vi "Main - Auto Detect Modules.vi"(8 "error in (no error)":errorcluster, 11 "Node Ptr":u64 format="%.0x") -> (0 "error out":errorcluster)   [LabVIEW 2020, in "SEECD System Explorer.lvlib"]
uses:
  SEECD System Explorer.lvlib
  Shared/Globals/String Constants.vi
  Shared/Globals/Scan Engine GUIDs.vi
  Shared/Globals/Property Strings.vi
  <vilib>/NI VeriStand/Custom Device API/Custom Device API.lvlib
  Shared/SEECD Shared.lvlib
  Scripting/Scan Engine Scripting.lvlib
panel:
  in  "Tag":string
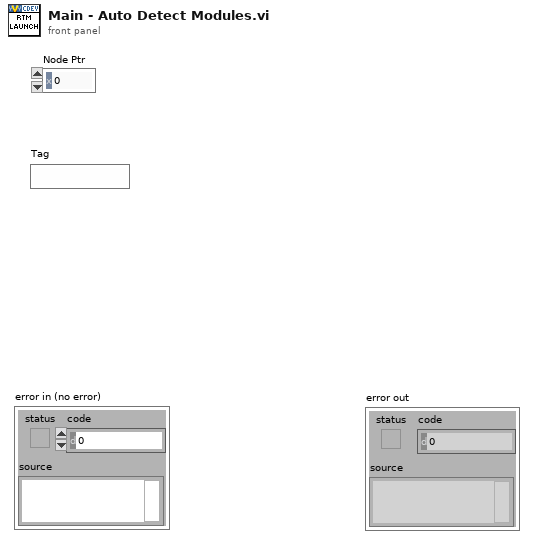
[diagram p1: front panel]
types:
  T1 = typedef "Custom Device API.lvlib/Custom Device Item Ref.ctl" = u64
  T2 = typedef "SEECD System Explorer.lvlib/Slot Programming Mode.ctl" = enum16{"Don't Modify", "Scan Engine", "LabVIEW FPGA", "NI-DAQmx"}
  T3 = typedef "SEECD System Explorer.lvlib/Host - HW Config.ctl" = cluster{"Local Chassis":T4, "Masters":T7[]}
  T4 = typedef "SEECD System Explorer.lvlib/Host - Local Chassis.ctl" = cluster{"Modules":T5[]}
  T5 = typedef "SEECD System Explorer.lvlib/Host - Module.ctl" = cluster{"IOV Ref":string, "Slot":u32, "Model":u32, "All Variables":T6[]}
  T6 = typedef "SEECD System Explorer.lvlib/IOV Container Contents.ctl" = cluster{"Name":string, "Writable":bool, "DataType":variant}
  T7 = typedef "SEECD System Explorer.lvlib/Host - Master.ctl" = cluster{"IOV Ref":string, "Name":string, "Master ID":u32, "Slaves":T8[]}
  T8 = typedef "SEECD System Explorer.lvlib/Host - Slave.ctl" = cluster{"IOV Ref":string, "Name":string, "Position Address":u16, "Bitfile Signature":u8[], "Modules":T5[], "ECAT IOV Contents":T6[]}
  T9 = typedef "Custom Device API.lvlib/Custom Device Item Info.ctl" = cluster{"Name":string, "Is Channel":bool, "GUID":string, "Is Waveform":bool}
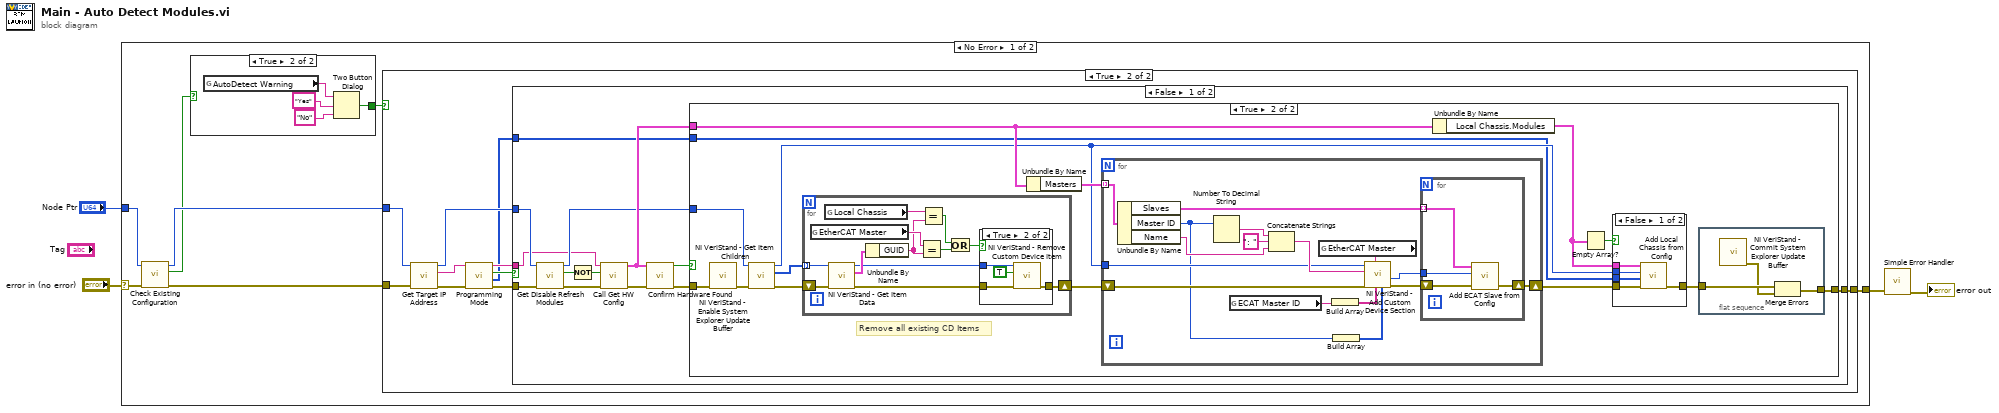
[diagram p0: block diagram]
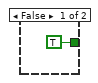
[diagram p7: hidden frame]
diagram:
  n1 = case shown="No Error" "error in (no error)" {
    selector: "error in (no error)" -> [w9 w104]
    tunnel: "Node Ptr" -> [w7 _]
    tunnel: [w10 w104] -> w2
    frame No Error {
      n2 = call "Check Existing Configuration.vi"("error in"=w9, "Item Ref in"=w7) -> ("error out"=w8:errorcluster, "Existing Configuration Exists"=w5:bool, "Item Ref out"=w6:T1)  [unwired: 7 in]
      n3 = case shown="True" w5 {
        tunnel: [TRUE ("T button?") w103] -> w11
        frame False {
        }
        frame True {
          n4 = global read "String Constants.vi" "AutoDetect Warning"() -> (w100:string)
          n5 = Two Button Dialog(message=w100, 1:"No" ("F button name (\"Cancel\")"), 2:"Yes" ("T button name (\"OK\")")) -> (T button?=w103:bool)
        }
      }
      n6 = case shown="True" w11 {
        tunnel: w8 -> [w12 w17]
        tunnel: [w12 w22] -> w10
        tunnel: w6 -> [_ w16]
        frame False {
        }
        frame True {
          n7 = call "Get Target IP Address.vi"("error in"=w17, "Item Ref in"=w16) -> ("error out"=w20:errorcluster, "Target IP Address"=w21:string, "Item Ref out"=w15:T1)  [unwired: 7 in]
          n8 = call "Programming Mode.vi"("error in (no error)"=w20, "serverName In"=w21) -> ("error out"=w18:errorcluster, "Programming Mode Out"=w13:T2[], "Cancelled"=w14:bool, "serverName Out"=w19:string)  [unwired: 6 in]
          n9 = case shown="False" w14 {
            tunnel: [w35 w98] -> w22
            tunnel: w19 -> [w23 _]
            tunnel: w18 -> [w29 w98]
            tunnel: w15 -> [w27 _]
            tunnel: w13 -> [w30 _]
            frame False {
              n10 = call "Get Disable Refresh Modules.vi"("error in"=w29, "scan engine custom device ref in"=w27) -> ("error out"=w28:errorcluster, "disable refresh modules"=w24:bool, "scan engine custom device ref out"=w26:T1)  [unwired: 7 in]
              n11 = Not(x=w24) -> (.not. x?=w25:bool)
              n12 = call "Call Get HW Config.vi"("error in"=w28, "Refresh Modules"=w25, "serverName"=w23) -> ("error out"=w32:errorcluster, "HW Config"=w34:T3)  [unwired: 7 in]
              n13 = call "Confirm Hardware Found.vi"("error in"=w32, "HW Config"=w34) -> ("error out"=w31:errorcluster, "Configure Hardware?"=w33:bool)  [unwired: 8 in]
              n14 = case shown="True" w33 {
                tunnel: w31 -> [w36 w41]
                tunnel: [w36 w46] -> w35
                tunnel: w34 -> [_ w45]
                tunnel: w26 -> [_ w39]
                tunnel: w30 -> [_ w37]
                frame False {
                }
                frame True {
                  # "Remove all existing CD Items"
                  n15 = call <vilib>:"NI VeriStand - Enable System Explorer Update Buffer.vi"("error in (no error)"=w41) -> ("error out"=w42:errorcluster)  [unwired: 10 in]
                  n16 = call <vilib>:"NI VeriStand - Get Item Children.vi"("error in (no error)"=w42, "Item Ref in"=w39) -> ("error out"=w43:errorcluster, "Child Refs"=w44:T1[], "Item Ref out"=w38:T1)  [unwired: 6 in, 1 out]
                  n17 = for {
                    tunnel: w44 -> [w92] mode=indexing
                    shift-right: [w86] -> w40
                    shift-left: w43 -> [w91]
                    n18 = global read "Scan Engine GUIDs.vi" "EtherCAT Master"() -> (w89:string)
                    n19 = global read "Scan Engine GUIDs.vi" "Local Chassis"() -> (w85:string)
                    n20 = call <vilib>:"NI VeriStand - Get Item Data.vi"("error in (no error)"=w91, "Item Ref in"=w92) -> ("error out"=w87:errorcluster, "Item Info"=w90:T9, "Item Ref out"=w88:T1)  [unwired: 6 in, 1 out]
                    n21 = Unbundle By Name(w90) -> ("GUID"=w84:string)
                    n22 = Equal?(x=w89, y=w84) -> (x = y?=w82:bool)
                    n23 = Equal?(x=w85, y=w84) -> (x = y?=w83:bool)
                    n24 = Or(x=w83, y=w82) -> (x .or. y?=w81:bool)
                    n25 = case shown="True" w81 {
                      tunnel: w88 -> [_ w96]
                      tunnel: w87 -> [w93 w97]
                      tunnel: [w93 w95] -> w86
                      frame False {
                      }
                      frame True {
                        n26 = call <vilib>:"NI VeriStand - Remove Custom Device Item.vi"("error in (no error)"=w97, "Force Delete (F)"=TRUE, "Item Ref in"=w96) -> ("error out"=w95:errorcluster)  [unwired: 7 in, 1 out]
                      }
                    }
                  }
                  n27 = Unbundle By Name(w45) -> ("Masters"=w51:T7[])
                  n28 = for {
                    tunnel: w51 -> [w71] mode=indexing
                    shift-right: [w61] -> w50
                    shift-left: w40 -> [w72]
                    tunnel: w38 -> [w73]
                    n29 = Unbundle By Name(w71) -> ("Slaves"=w63:T8[], "Master ID"=w66:u32, "Name"=w68:string)
                    n30 = Number To Decimal String(number=w66) -> (decimal integer string=w70:string)  [unwired: 1 in]
                    n31 = global read "Property Strings.vi" "ECAT Master ID"() -> (w67:string)
                    n32 = Concatenate Strings(w70, ": " ("string"), w68) -> (w74:string)
                    n33 = global read "Scan Engine GUIDs.vi" "EtherCAT Master"() -> (w76:string)
                    n34 = Build Array(w67) -> (w75:string[])
                    n35 = Build Array(w66) -> (w65:u32[])
                    n36 = call <vilib>:"NI VeriStand - Add Custom Device Section.vi"("Property Values"=w65, "Property names"=w75, "GUID (Default Section)"=w76, "error in (no error)"=w72, "Section Name"=w74, "Parent Ref in"=w73) -> ("error out"=w64:errorcluster, "Section Ptr"=w62:T1)  [unwired: 2 in, 2 out]
                    n37 = for {
                      shift-right: [w77] -> w61
                      shift-left: w64 -> [w79]
                      tunnel: w63 -> [w80] mode=indexing
                      tunnel: w62 -> [w78]
                      n38 = call "Add ECAT Slave from Config.vi"("error in (no error)"=w79, "Section Ptr"=w78, "Slave"=w80) -> ("error out"=w77:errorcluster)  [unwired: 8 in]
                    }
                  }
                  n39 = Unbundle By Name(w45) -> ("Local Chassis.Modules"=w49:T5[])
                  n40 = Empty Array?(array=w49) -> (empty?=w48:bool)
                  n41 = case shown="False" w48 {
                    tunnel: w50 -> [w59 w60]
                    tunnel: w38 -> [w58 _]
                    tunnel: w49 -> [w57 _]
                    tunnel: [w56 w60] -> w47
                    tunnel: w37 -> [w55 _]
                    frame False {
                      n42 = call "Add Local Chassis from Config.vi"("error in"=w59, "Programming Mode"=w55, "Item Ref in"=w58, "Modules"=w57) -> ("error out"=w56:errorcluster)  [unwired: 7 in]
                    }
                    frame True {
                    }
                  }
                  n43 = flat-sequence {
                    tunnel: w47 -> [w54]
                    tunnel: [w52] -> w46
                    frame #0 {
                      n44 = call <vilib>:"NI VeriStand - Commit System Explorer Update Buffer.vi"() -> ("error out"=w53:errorcluster)  [unwired: 11 in]
                      n45 = Merge Errors(w54, w53) -> (w52:errorcluster)
                    }
                  }
                }
              }
            }
            frame True {
            }
          }
        }
      }
    }
    frame Error {
    }
  }
  n46 = call <vilib>:"Simple Error Handler.vi"("error in (no error)"=w2) -> ("error out"=→"error out":errorcluster)  [unwired: 4 in, 4 out]
